vi "anal txt each save.vi"(5 "B Table":string[][](table), 6 "R Table":string[][](table), 7 "S Table":string[][](table), 8 "error in":errorcluster, 11 "Table Pass refnum_in":T1) -> (0 "error out":errorcluster, 3 "Table Pass refnum_out":T1)   [LabVIEW 2018]
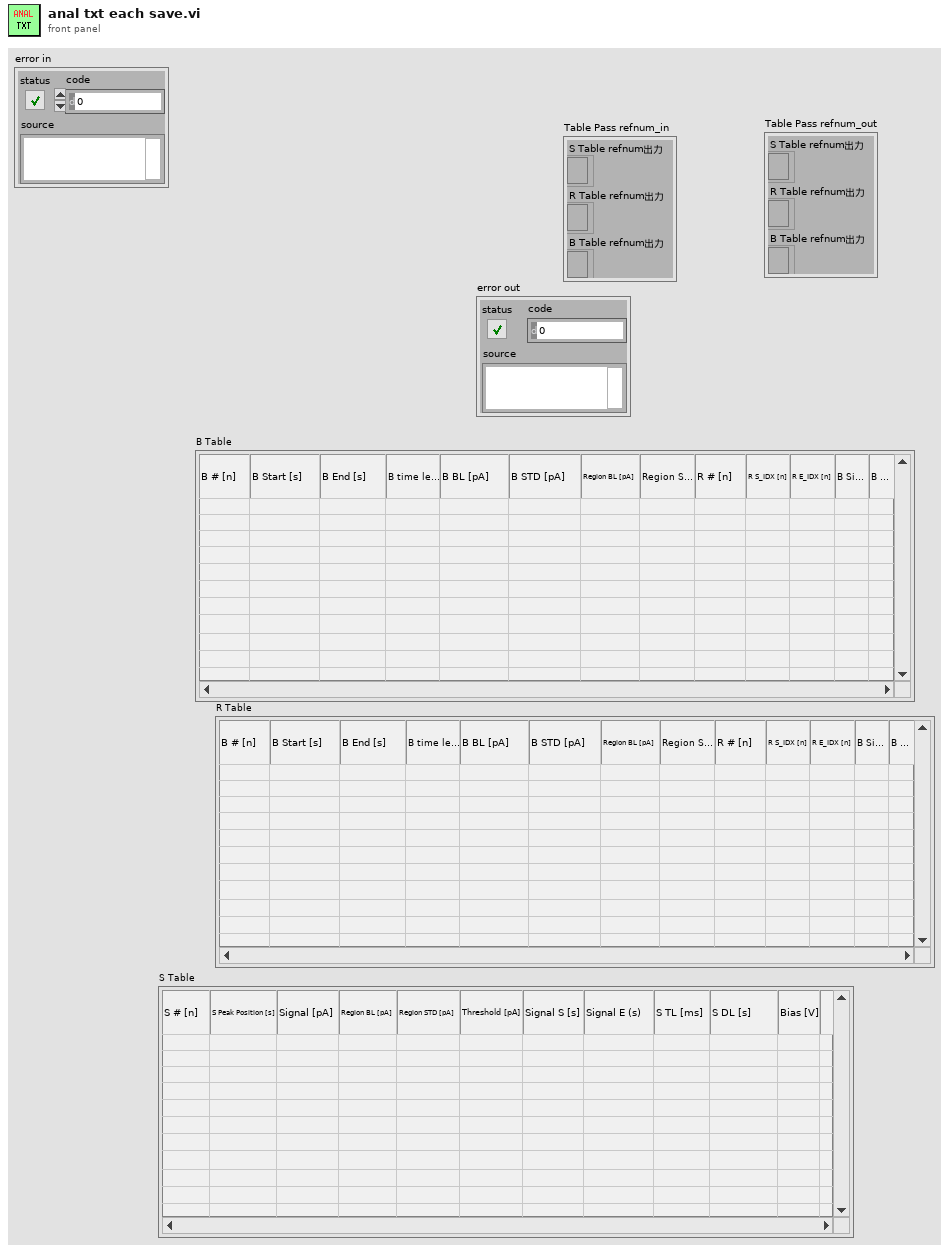
[diagram p1: front panel]
types:
  T1 = cluster{"S Table refnum出力":refnum<file>, "R Table refnum出力":refnum<file>, "B Table refnum出力":refnum<file>}
  T2 = cluster{"refnum out":refnum<file>, "refnum out":refnum<file>, "refnum out":refnum<file>}
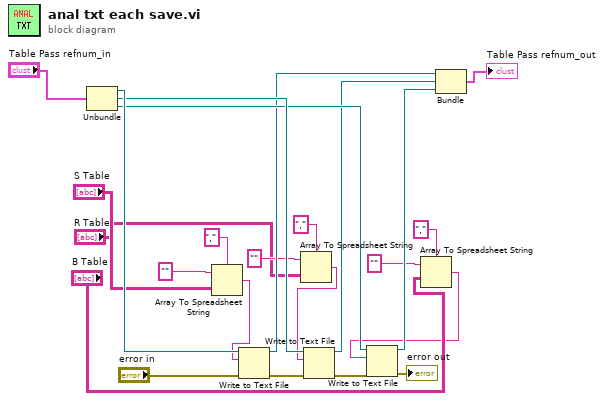
[diagram p0: block diagram]
diagram:
  n1 = Unbundle("Table Pass refnum_in") -> ("S Table refnum出力"=w19:refnum<file>, "R Table refnum出力"=w18:refnum<file>, "B Table refnum出力"=w17:refnum<file>)
  n2 = Array To Spreadsheet String(delimiter (Tab)="," ("デリミタ（タブ）"), array="S Table", 3:"" ("形式文字列")) -> (spreadsheet string=w9:string)
  n3 = Write to Text File(file (use dialog)=w19, text=w9, error in="error in") -> (refnum out=w15:refnum<file>, error out=w24:errorcluster)  [unwired: 1 in, 1 out]
  n4 = Array To Spreadsheet String(delimiter (Tab)="," ("デリミタ（タブ）"), array="R Table", 3:"" ("形式文字列")) -> (spreadsheet string=w3:string)
  n5 = Write to Text File(file (use dialog)=w18, text=w3, error in=w24) -> (refnum out=w14:refnum<file>, error out=w23:errorcluster)  [unwired: 1 in, 1 out]
  n6 = Array To Spreadsheet String(delimiter (Tab)="," ("デリミタ（タブ）"), array="B Table", 3:"" ("形式文字列")) -> (spreadsheet string=w1:string)
  n7 = Write to Text File(file (use dialog)=w17, text=w1, error in=w23) -> (refnum out=w13:refnum<file>, error out=→"error out":errorcluster)  [unwired: 1 in, 1 out]
  n8 = Bundle("refnum out"=w15, "refnum out"=w14, "refnum out"=w13) -> (→"Table Pass refnum_out":T2)  [unwired: 1 in]
